vi "Test_Setup.vi"(0 "Level":i32=1, 1 "Torch":bool, 2 "Phase":i32=2, 3 "Keys":i32, 5 "Room":i32=-1, 7 "X":i32, 9 "Y":i32, 11 "error in":errorcluster) -> (4 "State":T2={"Tick"=0, "Phase"=0, "PhaseTicks"=0, "Level"=1, "Room"=0, "X10"=0, "Y10"=0, "VY10"=0, "Mode"=0, "Facing"=0, "Run"=0, "Vert"=0, "StandY"=0, "EntryX10"=0, "EntryY10"=0, "EntryMode"=0, "Lives"=4, "Score"=0, "NextLife"=10000, "KeyR"=0, "KeyB"=0, "KeyY"=0, "Torch"=FALSE, "FloorPhase"=0, "Dead"=FALSE, "LevelStart"=FALSE, "Quit"=FALSE, "Sound"=0, "Seed"=12345, "DemoStep"=0, "Tiles"=[], "World"=[], "Enemies"=[], "Highscores"=[], "Name"=[0, 0, 0], "Cursor"=0}, 6 "Rooms":T1(array[cluster]), 15 "error out":errorcluster)   [LabVIEW 2026]
doc: "Test helper: Game_Start, then a new game in Level; with Room >= 0 Claude is put into that room at (X, Y) px (the room gets its tiles and enemies, the position is the restart point). Torch sets the torch, Keys the number of keys of each colour. Phase = phase to start in (2 = Playing)."
uses:
  Source/Engine/GH_Engine.lvlib
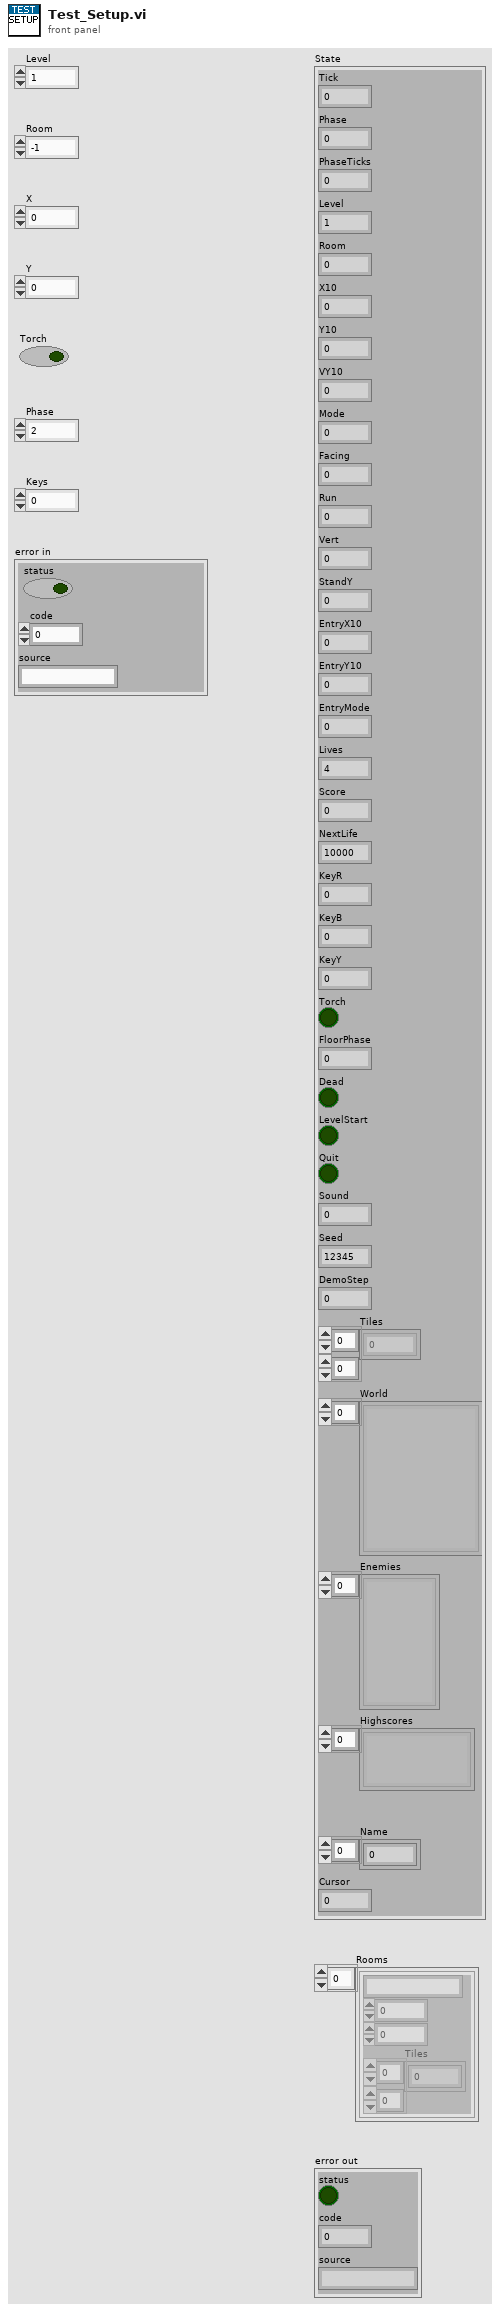
[diagram p1: front panel]
types:
  T1 = cluster{"ID":string, "Depth":i32, "Column":i32, "Tiles":u8[][]}[]
  T2 = cluster{"Tick":u32, "Phase":i32, "PhaseTicks":i32, "Level":i32, "Room":i32, "X10":i32, "Y10":i32, "VY10":i32, "Mode":i32, "Facing":i32, "Run":i32, "Vert":i32, "StandY":i32, "EntryX10":i32, "EntryY10":i32, "EntryMode":i32, "Lives":i32, "Score":i32, "NextLife":i32, "KeyR":i32, "KeyB":i32, "KeyY":i32, "Torch":bool, "FloorPhase":i32, "Dead":bool, "LevelStart":bool, "Quit":bool, "Sound":i32, "Seed":u32, "DemoStep":i32, "Tiles":u8[][], "World":cluster{"ID":string, "Depth":i32, "Column":i32, "Tiles":u8[][]}[], "Enemies":cluster{"Kind":i32, "X10":i32, "Y10":i32, "Dir":i32, "Mode":i32}[], "Highscores":cluster{"Score":i32, "Name":string}[], "Name":i32[], "Cursor":i32}
  T3 = cluster{"ID":string, "Depth":i32, "Column":i32, "Tiles":u8[][]}
  T4 = cluster{"Kind":i32, "X10":i32, "Y10":i32, "Dir":i32, "Mode":i32}[]
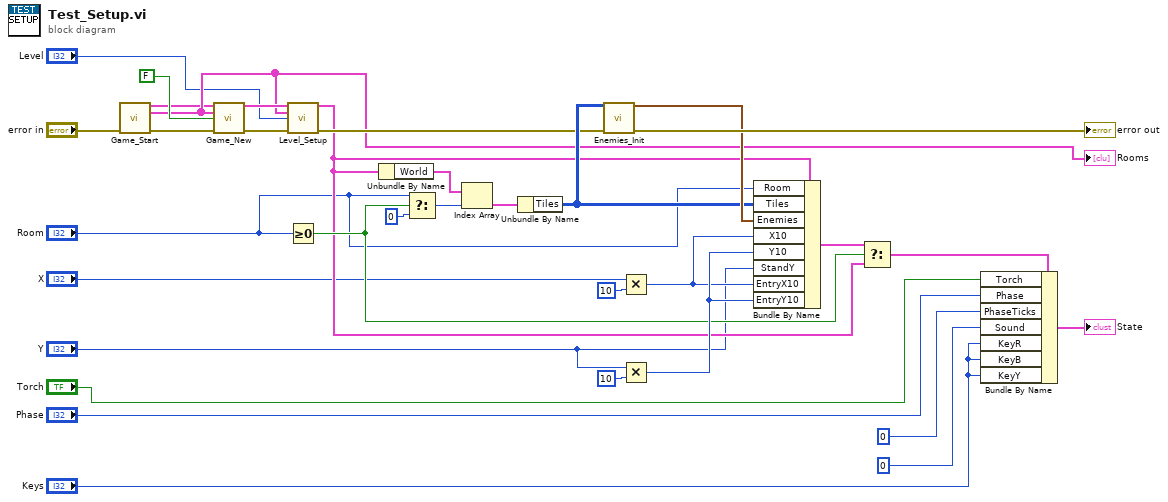
[diagram p0: block diagram]
diagram:
  n1 = call "Game_Start.vi"("error in"="error in") -> ("State"=w9:T2, "Rooms"=w10:T1, "error out"=w11:errorcluster)  [unwired: 12 in]
  "Rooms" <- w10
  n2 = call "Game_New.vi"("State"=w9, "Rooms"=w10, "Demo"=FALSE, "error in"=w11) -> ("State out"=w13:T2, "error out"=w14:errorcluster)  [unwired: 10 in]
  n3 = call "Level_Setup.vi"("State"=w13, "Rooms"=w10, "Level"="Level", "error in"=w14) -> ("State out"=w15:T2, "error out"=w16:errorcluster)  [unwired: 10 in]
  n4 = Greater Or Equal To 0?(x="Room") -> (x >= 0?=w18:bool)
  n5 = Unbundle By Name(w15) -> ("World"=w17:T1)
  n6 = Select(t="Room", s=w18, f=0) -> (s? t:f=w20:i32)
  n7 = Index Array(array=w17, index=w20) -> (element=w21:T3)
  n8 = Unbundle By Name(w21) -> ("Tiles"=w22:u8[][])
  n9 = call "Enemies_Init.vi"("Tiles"=w22, "error in"=w16) -> ("Enemies"=w23:T4, "error out"=→"error out":errorcluster)  [unwired: 12 in]
  n10 = Multiply(x="X", y=10) -> (x*y=w26:i32)
  n11 = Multiply(x="Y", y=10) -> (x*y=w28:i32)
  n12 = Bundle By Name(cluster=w15, "Room"="Room", "Tiles"=w22, "Enemies"=w23, "X10"=w26, "Y10"=w28, "StandY"="Y", "EntryX10"=w26, "EntryY10"=w28) -> (w29:T2)
  n13 = Select(t=w29, s=w18, f=w15) -> (s? t:f=w30:T2)
  n14 = Bundle By Name(cluster=w30, "Torch"="Torch", "Phase"="Phase", "PhaseTicks"=0, "Sound"=0, "KeyR"="Keys", "KeyB"="Keys", "KeyY"="Keys") -> (→"State":T2)
